vi "Stop Tick.vi"(11 "Actor in":refnum<class "VTU Sim Rig.lvclass">) -> (0 "error out":errorcluster, 3 "Actor out":refnum<class "VTU Sim Rig.lvclass">)   [LabVIEW 2026, in "VTU Sim Rig.lvclass"]
doc: "Stop Core hook (seriesAfter). Stops and releases the Time-Delayed Send delivery notifier held in Tick Notifier."
uses:
  C:/Users/DynaAdmin/PycharmProjects/Universal-sequence-executor-AF/plugins/VTU Sim Rig/VTU Sim Rig.lvclass
  C:/Users/DynaAdmin/PycharmProjects/Universal-sequence-executor-AF/plugins/VTU Sim Rig/VTU Sim Rig.lvclass/VTU Sim Rig.ctl
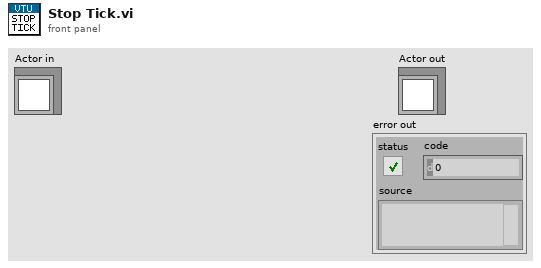
[diagram p1: front panel]
types:
  T1 = enum16{"Send next copy now", "Skip next scheduled copy", "Send next copy now and stop all further copies", "Stop all further copies"}
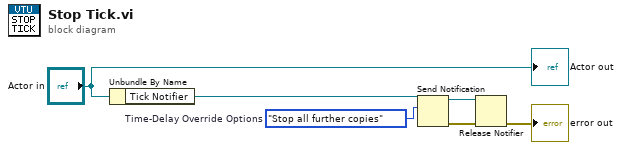
[diagram p0: block diagram]
diagram:
  w5 = T1."Stop all further copies"  # Time-Delay Override Options
  n1 = Unbundle By Name("Actor in") -> ("Tick Notifier"=w6:refnum<notifier>)
  n2 = Send Notification(notification=w5, notifier=w6) -> (notifier out=w4:refnum<notifier>, error out=w3:errorcluster)  [unwired: 1 in]
  n3 = Release Notifier(notifier=w4, error in (no error)=w3) -> (error out=→"error out":errorcluster)  [unwired: 1 in, 2 out]
  "Actor out" <- "Actor in"
